vi "Add Control to Server ClusterDef.vi"(5 "New Control Label":string, 6 "Clear Previous ?(F)":bool, 7 "Source Control ref in":refnum<vi>, 8 "error in (no error)":errorcluster, 10 "Target ClusterDef Name":string, 11 "Server class in":refnum<vi>) -> (0 "error out":errorcluster, 3 "Server class out":refnum<vi>)   [LabVIEW 2019, in "gRPC Template Creation Utility.lvlib"]
uses:
  gRPC Template Creation Utility.lvlib
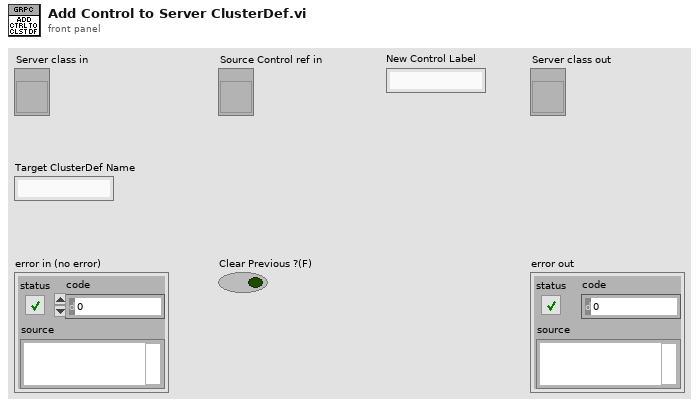
[diagram p1: front panel]
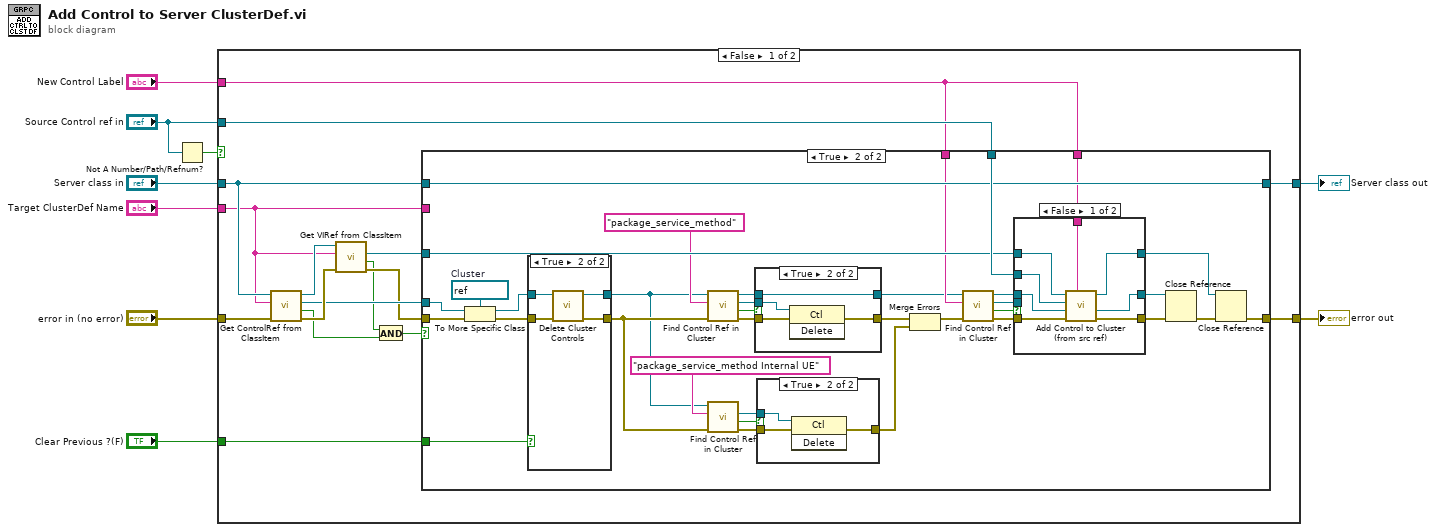
[diagram p0: block diagram]
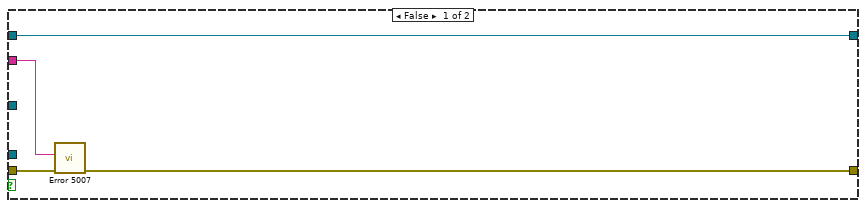
[diagram p2: hidden frame]
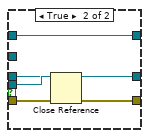
[diagram p3: hidden frame]
diagram:
  n1 = Not A Number/Path/Refnum?(number/path/refnum="Source Control ref in") -> (NaN/Path/Refnum?=w1:bool)
  n2 = case shown="False" w1 {
    tunnel: [w25 w94] -> w9
    tunnel: "Target ClusterDef Name" -> [w10 _]
    tunnel: "error in (no error)" -> [w20 w94]
    tunnel: "New Control Label" -> [w11 _]
    tunnel: "Server class in" -> [w15 w95]
    tunnel: [w14 w95] -> w4
    tunnel: "Clear Previous ?(F)" -> [w13 _]
    tunnel: "Source Control ref in" -> [w12 _]
    frame False {
      n3 = call "Get ControlRef from ClassItem.vi"("error in (no error)"=w20, "Item Name"=w10, "LVClassLibrary in"=w15) -> ("error out"=w22:errorcluster, "Found ?"=w18:bool, "Control ref out"=w21:refnum<vi>, "LVClassLibrary out"=w23:refnum<vi>)  [unwired: 5 in]
      n4 = call "Get VIRef from ClassItem.vi"("error in (no error)"=w22, "Item Name"=w10, "LVClassLibrary in"=w23) -> ("error out"=w19:errorcluster, "Found ?"=w17:bool, "VIref out"=w24:refnum<vi>)  [unwired: 5 in, 1 out]
      n5 = And(x=w17, y=w18) -> (x .and. y?=w16:bool)
      n6 = case shown="True" w16 {
        tunnel: [w27 w32] -> w25
        tunnel: w12 -> [_ w64]
        tunnel: w24 -> [_ w63]
        tunnel: w21 -> [_ w62]
        tunnel: w19 -> [w28 w60]
        tunnel: w15 -> [w29 w59]
        tunnel: [w29 w59] -> w14
        tunnel: w13 -> [_ w56]
        tunnel: w11 -> [_ w42]
        tunnel: w11 -> [_ w37]
        tunnel: w10 -> [w26 _]
        frame False {
          n7 = call "Error 5007.vi"("error in (no error)"=w28, "Target ClusterDef Name"=w26) -> ("error out"=w27:errorcluster)  [unwired: 9 in]
        }
        frame True {
          w61 = refnum<vi> refnum  # Cluster
          n8 = To More Specific Class(target class=w61, reference=w62, error in=w60) -> (specific class reference=w58:refnum<vi>, error out=w57:errorcluster)
          n9 = case shown="True" w56 {
            tunnel: w58 -> [w89 w93]
            tunnel: w57 -> [w88 w92]
            tunnel: [w89 w91] -> w46
            tunnel: [w88 w90] -> w47
            frame False {
            }
            frame True {
              n10 = call "Delete Cluster Controls.vi"("error in (no error)"=w92, "Cluster in"=w93) -> ("error out"=w90:errorcluster, "Cluster out"=w91:refnum<vi>)  [unwired: 8 in]
            }
          }
          n11 = call "Find Control Ref in Cluster.vi"("error in (no error)"=w47, "Control Name"="package_service_method", "Cluster ref in"=w46) -> ("error out"=w52:errorcluster, "Found ?"=w54:bool, "Ctl ref"=w53:refnum<vi>, "Cluster ref out"=w31:refnum<vi>)  [unwired: 5 in]
          n12 = call "Find Control Ref in Cluster.vi"("error in (no error)"=w47, "Control Name"="package_service_method Internal UE", "Cluster ref in"=w46) -> ("error out"=w51:errorcluster, "Found ?"=w49:bool, "Ctl ref"=w50:refnum<vi>)  [unwired: 5 in, 1 out]
          n13 = case shown="True" w54 {
            tunnel: w53 -> [_ w87]
            tunnel: w52 -> [w83 w86]
            tunnel: [w83 w85] -> w45
            tunnel: w31 -> [w82 w84]
            tunnel: [w82 w84] -> w30
            frame False {
            }
            frame True {
              n14 = invoke class="Ctl" method="Delete"(reference=w87, error in=w86) -> (error out=w85:errorcluster)  [unwired: 1 in, 2 out]
            }
          }
          n15 = case shown="True" w49 {
            tunnel: w50 -> [_ w81]
            tunnel: w51 -> [w78 w80]
            tunnel: [w78 w79] -> w44
            frame False {
            }
            frame True {
              n16 = invoke class="Ctl" method="Delete"(reference=w81, error in=w80) -> (error out=w79:errorcluster)  [unwired: 1 in, 2 out]
            }
          }
          n17 = Merge Errors(w45, w44) -> (w43:errorcluster)
          n18 = call "Find Control Ref in Cluster.vi"("error in (no error)"=w43, "Control Name"=w42, "Cluster ref in"=w30) -> ("error out"=w40:errorcluster, "Found ?"=w39:bool, "Ctl ref"=w38:refnum<vi>, "Cluster ref out"=w41:refnum<vi>)  [unwired: 5 in]
          n19 = case shown="False" w39 {
            tunnel: [w68 w75] -> w35
            tunnel: w64 -> [w72 _]
            tunnel: w63 -> [w71 w73]
            tunnel: w41 -> [w70 w74]
            tunnel: w40 -> [w69 w76]
            tunnel: w38 -> [_ w77]
            tunnel: w37 -> [w67 _]
            tunnel: [w65 w74] -> w34
            tunnel: [w66 w73] -> w33
            frame False {
              n20 = call "Add Control to Cluster (from src ref).vi"("New Control Label"=w67, "error in (no error)"=w69, "Cluster ref in (owner)"=w70, "Source control ref in"=w72, "Owning VI ref in"=w71) -> ("error out"=w68:errorcluster, "Cluster ref out (owner)"=w65:refnum<vi>, "Owning VI ref out"=w66:refnum<vi>)  [unwired: 3 in, 1 out]
            }
            frame True {
              n21 = Close Reference(reference=w77, error in (no error)=w76) -> (error out=w75:errorcluster)
            }
          }
          n22 = Close Reference(reference=w34, error in (no error)=w35) -> (error out=w36:errorcluster)
          n23 = Close Reference(reference=w33, error in (no error)=w36) -> (error out=w32:errorcluster)
        }
      }
    }
    frame True {
    }
  }
  "error out" <- w9
  "Server class out" <- w4
